vi "Destroy.vi"(8 "error in (no error)":errorcluster, 11 "Camera in":refnum<class "Camera.lvclass">) -> (0 "error out":errorcluster)   [LabVIEW 2020, in "Camera.lvclass"]
doc: "Destroy the camera instance, aborting any streaming operation and freeing any associated resources."
uses:
  Camera.lvclass
  Camera.lvclass/Camera.ctl
  Check Not Disconnected.vi
  Check Stream OK.vi
  <vilib>/Utility/error.llb/Error Cluster From Error Code.vi
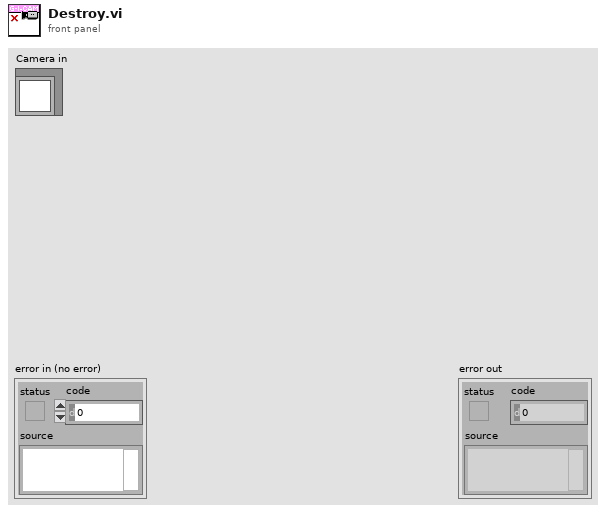
[diagram p1: front panel]
types:
  T1 = typedef "Camera.lvclass/Streaming Registation.ctl" = cluster{"Streaming Events":refnum<event-registration>, "User Events":T2}
  T2 = typedef "Camera.lvclass/Stream User Events.ctl" = cluster{"Stopped":refnum<user-event>, "Errors":refnum<user-event>}
  T3 = typedef "Camera.lvclass/Disconnected Registration.ctl" = cluster{"Disconnected":refnum<event-registration>, "User Event":refnum<user-event>}
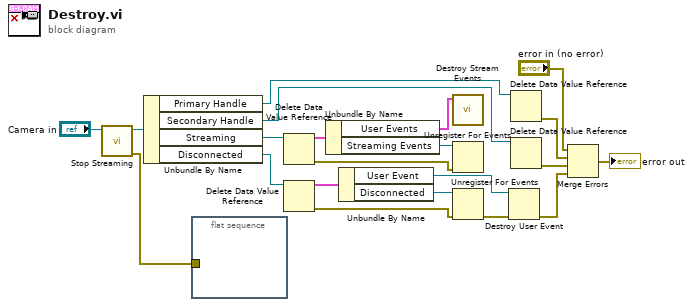
[diagram p0: block diagram]
diagram:
  n1 = call "Stop Streaming.vi"("Camera in"="Camera in") -> ("error out"=w1:errorcluster, "Camera"=w2:refnum<class "Camera.lvclass">)  [unwired: 9 in]
  n2 = Unbundle By Name(w2) -> ("Primary Handle"=w20:refnum<data-value>, "Secondary Handle"=w4:refnum<data-value>, "Streaming"=w16:refnum<data-value>, "Disconnected"=w13:refnum<data-value>)
  n3 = flat-sequence {
    tunnel: w1 -> [_]
    frame #0 {
    }
  }
  n4 = Delete Data Value Reference(data value reference=w16) -> (data value=w14:T1, error out=w15:errorcluster)  [unwired: 1 in]
  n5 = Delete Data Value Reference(data value reference=w13) -> (data value=w11:T3, error out=w7:errorcluster)  [unwired: 1 in]
  n6 = Unbundle By Name(w14) -> ("User Events"=w5:T2, "Streaming Events"=w12:refnum<event-registration>)
  n7 = Unbundle By Name(w11) -> ("User Event"=w9:refnum<user-event>, "Disconnected"=w8:refnum<event-registration>)
  n8 = call "Destroy Stream Events.vi"("Stream User Events"=w5) -> ()  [unwired: 10 in, 1 out]
  n9 = Unregister For Events(event registration refnum=w12, error in=w15) -> ()  [unwired: 1 out]
  n10 = Unregister For Events(event registration refnum=w8, error in=w7) -> (error out=w10:errorcluster)
  n11 = Destroy User Event(user event=w9, error in=w10) -> (error out=w6:errorcluster)
  n12 = Delete Data Value Reference(data value reference=w20) -> (error out=w19:errorcluster)  [unwired: 1 in, 1 out]
  n13 = Delete Data Value Reference(data value reference=w4) -> (error out=w3:errorcluster)  [unwired: 1 in, 1 out]
  n14 = Merge Errors("error in (no error)", w19, w3, w6) -> (→"error out":errorcluster)
